vi "FuncVI-vhShowCx.vi"(5 "InstanceRef":T2, 9 "arg list":T1[](array[typedef])) -> (0 "error out":bool, 3 "result":T1)   [LabVIEW 2021]
doc: "::: CalcExpress Toolkit :::\nCopyright (c) 2000-2026 Konstantin Shifershteyn. All rights reserved."
uses:
  cetypes.llb/CalcExpress Function Argument Info.ctl
  cetypes.llb/CalcExpress Instance RefNum.ctl
panel:
  in  "max arg num":i32=5
  in  "min arg num":i32=1
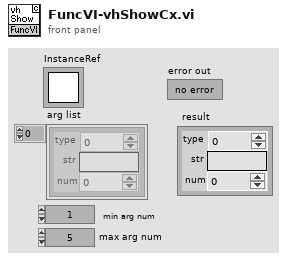
[diagram p1: front panel]
types:
  T1 = typedef "CalcExpress Function Argument Info.ctl" = cluster{"type":u32, "str":string, "num":dbl}
  T2 = typedef "CalcExpress Instance RefNum.ctl" = refnum<k1>
  T3 = cluster{"index":i32, "data type":enum32{"String", "DBL Number", "identifier", "1D Array of DBL", "2D Array of DBL", "CDB Number", "1D Array of CDB", "2D Array of CDB", "1D Array of String", "2D Array of String", "Unknown data type"}, "default num":dbl, "default str":string}[]
  T4 = cluster{"index":i32, "data type":enum32{"String", "DBL Number", "identifier", "1D Array of DBL", "2D Array of DBL", "CDB Number", "1D Array of CDB", "2D Array of CDB", "1D Array of String", "2D Array of String", "Unknown data type"}, "default num":dbl, "default str":string}
  T5 = cluster{"data type":enum32{"String", "DBL Number", "identifier", "1D Array of DBL", "2D Array of DBL", "CDB Number", "1D Array of CDB", "2D Array of CDB", "1D Array of String", "2D Array of String", "Unknown data type"}, "str":string, "num":dbl}
  T6 = typedef "VarMan Variable Context Handle.ctl" = i32
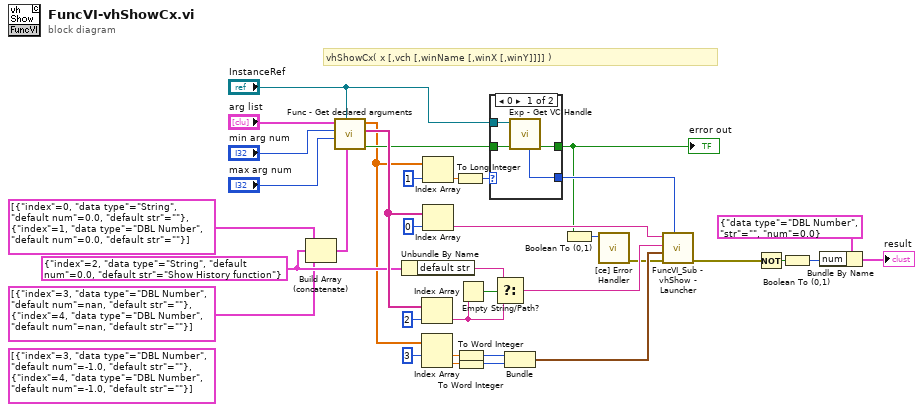
[diagram p0: block diagram]
diagram:
  (unwired) T3 [{"index"=3, "data type"=enum."DBL Number", "default num"=-1.0, "default str"=""}, {"index"=4, "data type"=enum."DBL Number", "default num"=-1.0, "default str"=""}]
  w29 = T4 {"index"=2, "data type"=enum."String", "default num"=0.0, "default str"="Show History function"} ("arg descriptor")
  # "vhShowCx( x [,vch [,winName [,winX [,winY]]]] )"
  n1 = Build Array (concatenate)(T3 [{"index"=0, "data type"=enum."String", "default num"=0.0, "default str"=""}, {"index"=1, "data type"=enum."DBL Number", "default num"=0.0, "default str"=""}], w29, T3 [{"index"=3, "data type"=enum."DBL Number", "default num"=nan, "default str"=""}, {"index"=4, "data type"=enum."DBL Number", "default num"=nan, "default str"=""}]) -> (w36:T3)
  n2 = call "Func - Get declared arguments.vi"("arg descriptors"=w36, "InstanceRef"="InstanceRef", "max arg num"="max arg num", "min arg num"="min arg num", "arg list"="arg list") -> ("error out"=w16:bool, "str list"=w33:string[], "num list"=w8:dbl[])  [unwired: 3 in, 1 out]
  n3 = Unbundle By Name(w29) -> ("default str"=w30:string)
  n4 = Index Array(array=w33, index=2) -> (element=w32:string)
  n5 = Index Array(array=w8, index #1=3) -> (element #1=w22:dbl, element #2=w1:dbl)  [unwired: 1 in]
  n6 = Index Array(array=w8, index=1) -> (element=w7:dbl)
  n7 = Index Array(array=w33, index=0) -> (element=w12:string)
  n8 = To Long Integer(number=w7) -> (32bit integer=w6:i32)
  n9 = To Word Integer(number=w22) -> (16bit integer=w21:i16)
  n10 = To Word Integer(number=w1) -> (16bit integer=w20:i16)
  n11 = Empty String/Path?(string/path=w32) -> (empty?=w31:bool)
  n12 = case shown="0" w6 {
    selector: w6 -> [_ w42]
    tunnel: w16 -> [w40 w41]
    tunnel: "InstanceRef" -> [w39 _]
    tunnel: [w38 w42] -> w14
    tunnel: [w37 w41] -> w3
    frame 0 {
      n13 = call "Exp - Get VC Handle.vi"("error in"=w40, "InstanceRef"=w39) -> ("error out"=w37:bool, "VC Handle"=w38:T6)  [unwired: 4 in, 2 out]
    }
    frame Default {
    }
  }
  "error out" <- w3
  n14 = Select(t=w30, s=w31, f=w32) -> (s? t:f=w28:string)
  n15 = Bundle(w21, w20) -> (w11:cluster{i16, i16})  [unwired: 1 in]
  n16 = Boolean To (0,1)(Boolean=w3) -> (0, 1=w5:i16)
  n17 = call "[ce] Error Handler.vi"("error code"=w5) -> ("error out"=w4:errorcluster)  [unwired: 9 in, 1 out]
  n18 = call "FuncVI_Sub - vhShow - Launcher.vi"("VC Handle"=w14, "error in"=w4, "left-top corner"=w11, "win name"=w28, "var name"=w12) -> ("error out"=w2:errorcluster)  [unwired: 6 in]
  n19 = Not(x=w2) -> (.not. x?=w17:bool)
  n20 = Boolean To (0,1)(Boolean=w17) -> (0, 1=w27:i16)
  n21 = Bundle By Name(cluster=T5 {"data type"=enum."DBL Number", "str"="", "num"=0.0} ("opd info"), "num"=w27) -> (→"result":T5)
